vi "GOOP_LVClass_Item_OnCommand.vi"(10 "Command Tag":string, 11 "Object":u64) -> ()   [LabVIEW 2020]
uses:
  <resource>/Framework/Providers/Open_GDS/SubVIs/GOOP_ClassProviderClassType.ctl
  <resource>/Framework/Providers/Open_GDS/ClassProviders/Provider_BaseClassInterface/ClassWriter_class/ClassWriter.lvclass
  <resource>/Framework/Providers/Open_GDS/ClassProviders/Common/ScriptingFunctions/Scripting_ConnectorPanePatternType.ctl
  <resource>/Framework/Providers/Open_GDS/SubVIs/GOOP_UMLEditor_CallMainAction.ctl
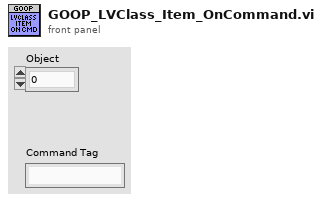
[diagram p1: front panel]
types:
  T1 = typedef "GOOP_ClassProviderClassType.ctl" = enum16{"ClassWriter", "ClassReader"}
  T2 = typedef "GOOP_UMLEditor_CallMainAction.ctl" = enum16{"OpenUmlEditor", "ReverseEngineering:WholeProject", "ReverseEngineering:OneClass", "ReverseEngineering:OneVI", "ShowInStateDiagram:OneVI", "OpenUMLFile"}
  T3 = enum8{"No dynamic dispatch VIs", "Include nearest implementation", "Include all overrides"}
  T4 = typedef "Scripting_ConnectorPanePatternType.ctl" = u16
  T5 = typedef "GDSLvCLass_ClassSettingsType.ctl" = cluster{"ClassProviderName":string, "ClassTemplateUsed":string, "ClassTemplateVersion":string, "ClassDescription":string, "PlugIns":T6[], "ConnectorPanePattern":string}
  T6 = typedef "GDSLvClass_PlugIn.ctl" = cluster{"Type":T7, "ID":string, "Version":string, "Path":path, "Name":string, "Data":variant}
  T7 = typedef "GDSLvClass_PlugInTypes.ctl" = enum16{"DesignPattern", "MethodTypes"}
  T8 = typedef "AddDesignPatternData.ctl" = cluster{"Type":string, "ID":string, "Version":string, "VIPath":path, "Name":string, "Data":variant}
  T9 = typedef "ClassWriter.lvclass/CreateMethodData.ctl" = cluster{"MethodName":string, "RelativeMethodPath":path, "MethodDescription":string, "Scope/Visibility":T10, "MethodTemplateName":string, "IconOut":u8[][], "RelativeProjectClassPath":string, "OpenViAfterCreation":bool, "DynamicDispatchVi":bool, "ExtraCreateParameters":variant, "MustOverride":bool, "MustCallParent":bool, "IconDetails":T11, "AF-Option":variant, "TemplatePath":path}
  T10 = typedef "GOOP300_MethodScopeType.ctl" = enum16{"Use Parent Folder Scope", "Public", "Protected", "Private", "Community"}
  T11 = typedef "ClassWriterNative.lvclass/IconDetails.ctl" = cluster{"IconSize":T12, "ImageRows(32)":i32, "ConnectorPaneHeight":i32[]}
  T12 = typedef "ClassWriterNative.lvclass/IconSize.ctl" = enum16{"Full", "1 c-term high", "2 c-term high", "3 c-term high"}
  T13 = typedef "ClassWriter.lvclass/CreateClassData.ctl" = cluster{"ClassName":string, "ClassFolder":path, "ClassDescription":string, "ClassTemplateOptions":string, "BaseClass(ProjectStringPath or LvClassFilePath)":variant, "ExtraCreateParameters":variant, "FolderSuffix":string, "ParentInterfaces":path[]}
  T14 = typedef "ItemRef.ctl" = u64
  T15 = typedef "ClassWriter.lvclass/HandleInterfacesData.ctl" = cluster{"InterfaceToAdd(Path)":path[], "InterfaceToRemove(Path)":path[], "MethodsToAddPerInterface(Empty=>All)":cluster{"InterfacePath":path, "Methods":string[]}[], "MethodsToRemovePerInterface(Empty=>All)":cluster{"InterfacePath":path, "Methods":string[]}[]}
  T16 = enum32{"invalid scope", "public", "private", "protected", "community"}
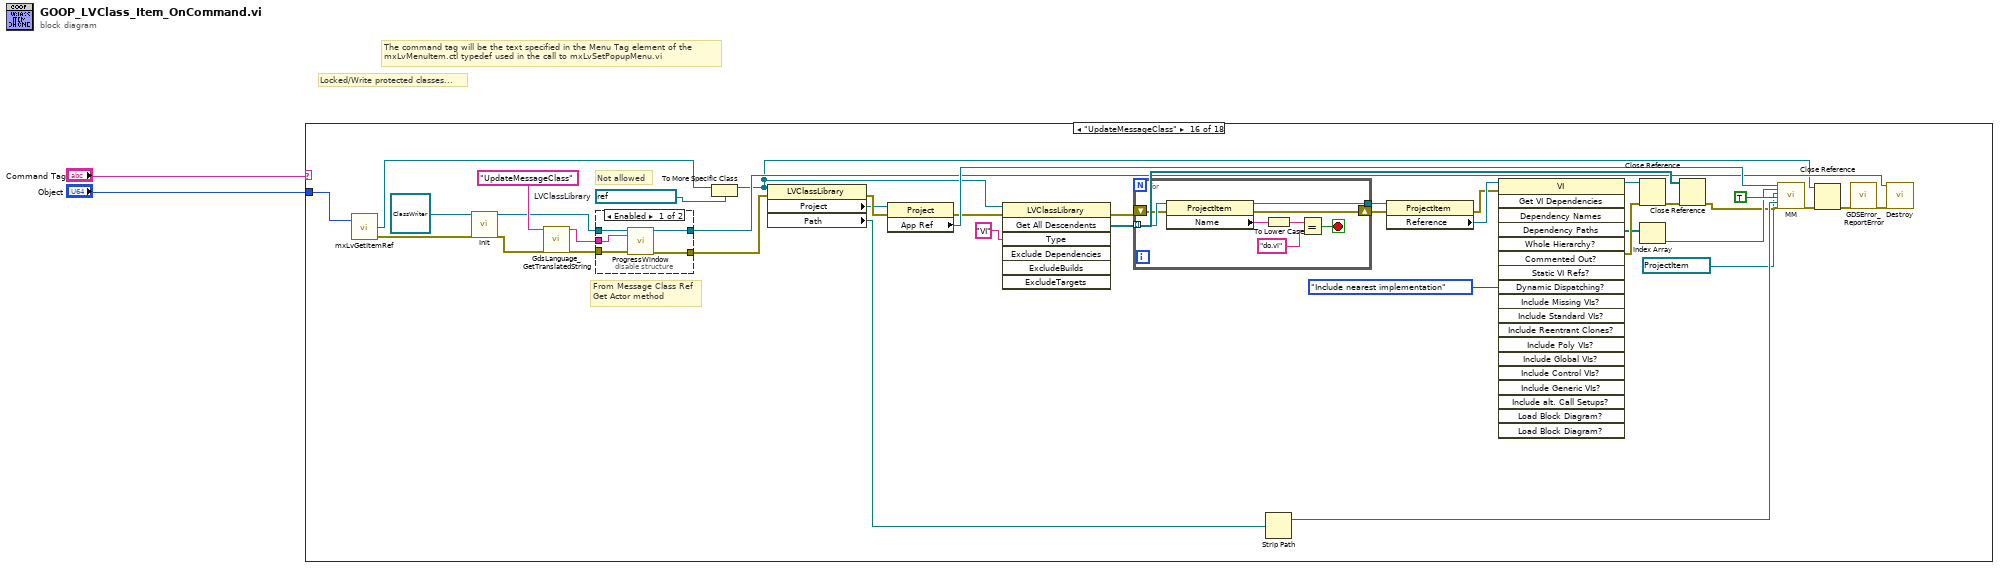
[diagram p0: block diagram]
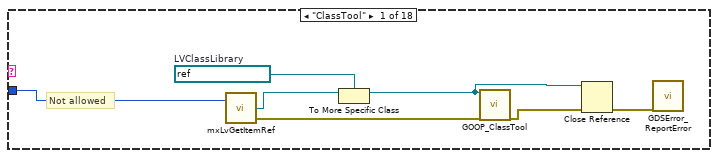
[diagram p2: hidden frame]
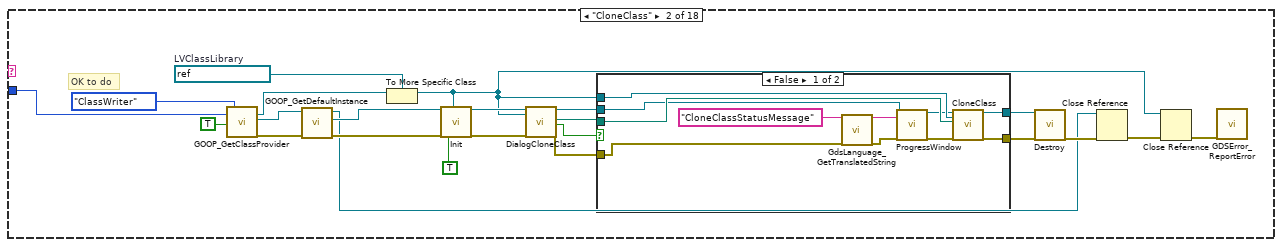
[diagram p3: hidden frame]
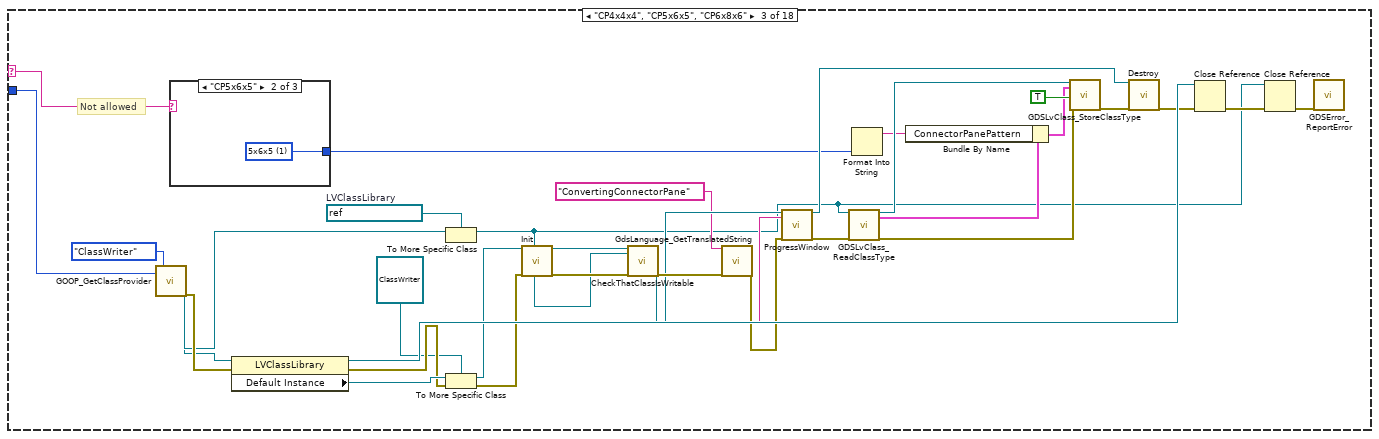
[diagram p5: hidden frame]
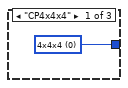
[diagram p6: hidden frame]
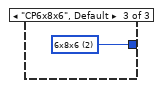
[diagram p7: hidden frame]
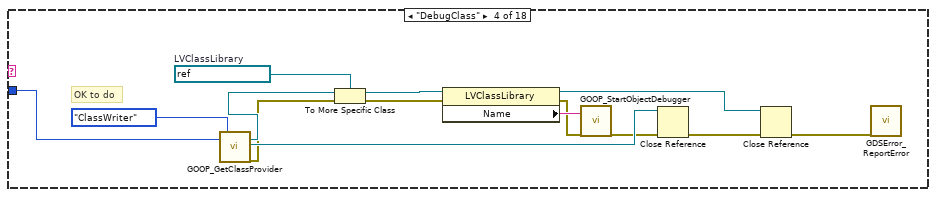
[diagram p8: hidden frame]
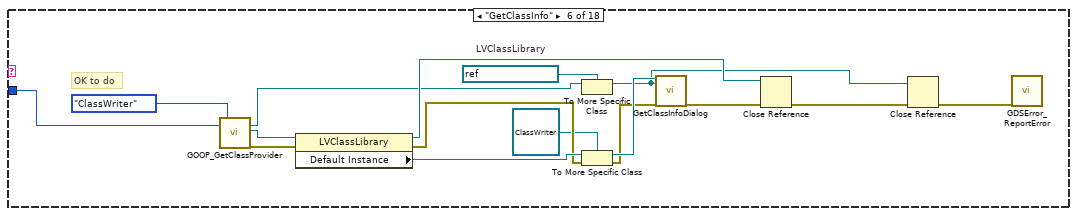
[diagram p10: hidden frame]
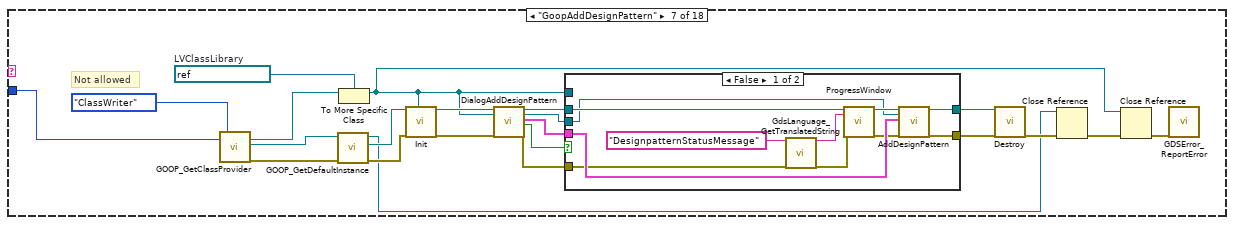
[diagram p11: hidden frame]
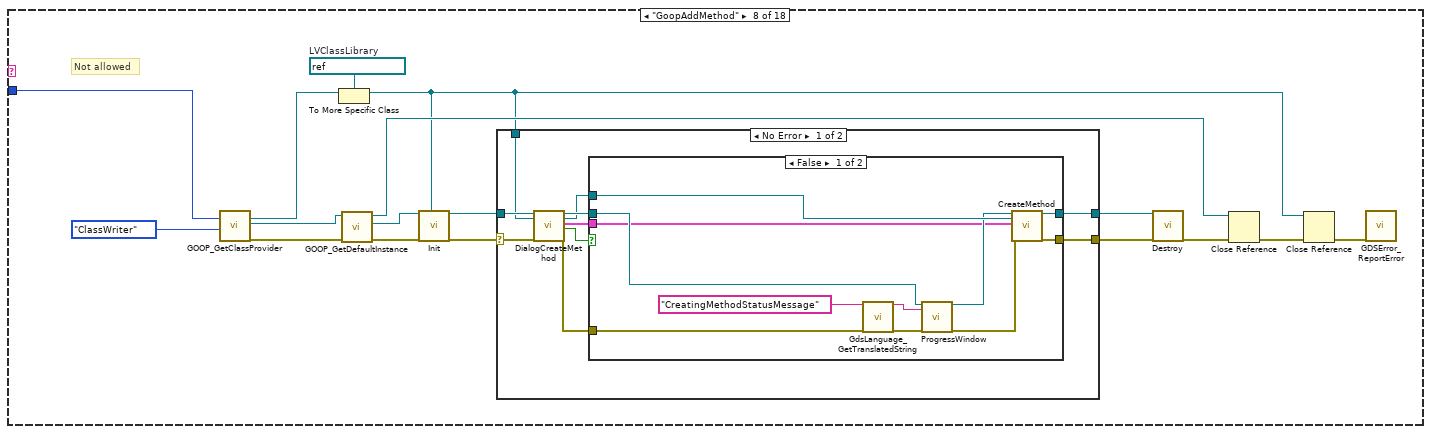
[diagram p13: hidden frame]
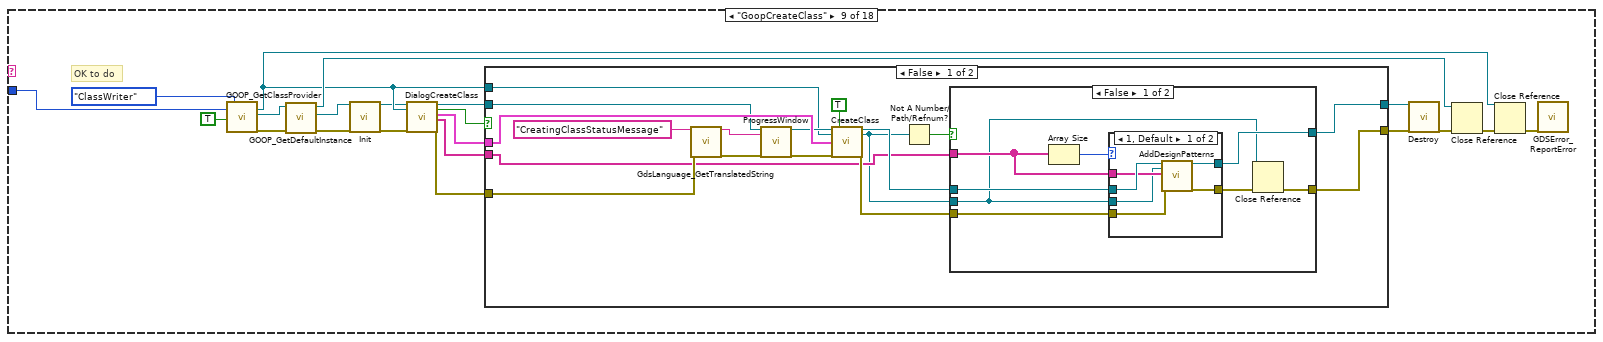
[diagram p16: hidden frame]
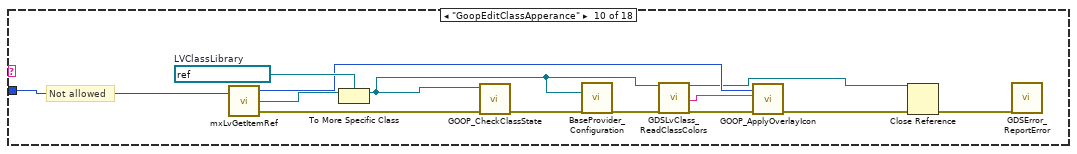
[diagram p20: hidden frame]
diagram:
  # "Locked/Write protected classes..."
  # "The command tag will be the text specified in the Menu Tag element of the \nmxLvMenuItem.ctl typedef used in the call to mxLvSetPopupMenu.vi"
  n1 = case shown="\"UpdateMessageClass\"" "Command Tag" {
    selector: "Command Tag" -> [_ _ w46 _ _ _ _ _ _ _ _ _ _ _ _ _ _ w522]
    tunnel: "Object" -> [w8 w19 w66 w83 _ w112 w134 w164 w210 w258 w268 w285 w323 w347 w373 w451 w470 w523]
    frame "ClassTool" {
      w9 = refnum<vi> refnum  # LVClassLibrary
      # "Not allowed"
      n2 = call <resource>:"mxLvGetItemRef.vi"("Item"=w8) -> ("Item Refnum"=w7:refnum<vi>, "error out"=w5:errorcluster)  [unwired: 1 in, 1 out]
      n3 = To More Specific Class(target class=w9, reference=w7) -> (specific class reference=w4:refnum<vi>)  [unwired: 1 in, 1 out]
      n4 = call <resource>:"GOOP_ClassTool.vi"("ClassRef"=w4, "Error In"=w5) -> ("Error Out"=w3:errorcluster)  [unwired: 17 in]
      n5 = Close Reference(reference=w4, error in (no error)=w3) -> (error out=w6:errorcluster)
      n6 = call <resource>:"GDSError_ReportError.vi"("error in (no error)"=w6) -> ()  [unwired: 18 in, 1 out]
    }
    frame "CloneClass" {
      w29 = refnum<vi> refnum  # LVClassLibrary
      # "OK to do"
      n7 = call <resource>:"GOOP_GetClassProvider.vi"("New Item Parent/Object"=w19, "CreateClass"=TRUE, "ProviderClassType"=GOOP_ClassProviderClassType."ClassWriter") -> ("ProjectItem"=w30:refnum<vi>, "LVClass.Open"=w16:refnum<vi>, "error out"=w17:errorcluster)  [unwired: 14 in]
      n8 = call <resource>:"GOOP_GetDefaultInstance.vi"("error in"=w17, "LVClassIn"=w16) -> ("error out"=w14:errorcluster, "ClassWriter.lvclass"=w15:refnum<class "ClassWriter.lvclass">, "LVClassOut"=w13:refnum<vi>)  [unwired: 7 in]
      n9 = To More Specific Class(target class=w29, reference=w30) -> (specific class reference=w10:refnum<vi>)  [unwired: 1 in, 1 out]
      n10 = call-dynamic "Init.vi"("ClassWriter in"=w15, "error in (no error)"=w14, "ClassFileMayBeReadOnly(False)"=TRUE, "LVClassLibrary Refnum"=w10) -> ("ClassWriter out"=w22:refnum<class "ClassWriter.lvclass">, "error out"=w21:errorcluster)  [unwired: 14 in]
      n11 = call-dynamic "DialogCloneClass.vi"("ClassWriter.lvclass"=w22, "ClassItemRefIn"=w10, "error in (no error)"=w21) -> ("ClassWriter.lvclassOut"=w27:refnum<class "ClassWriter.lvclass">, "NewClassPath"=w23:path, "Cancelled"=w24:bool, "error out"=w26:errorcluster)  [unwired: 12 in, 1 out]
      n12 = case shown="False" w24 {
        tunnel: w27 -> [w35 w44]
        tunnel: w26 -> [w36 w45]
        tunnel: [w40 w45] -> w25
        tunnel: w10 -> [w43 _]
        tunnel: w23 -> [w42 _]
        tunnel: [w41 w44] -> w20
        frame False {
          n13 = call <resource>:"GdsLanguage_GetTranslatedString.vi"("StringID(s)"="CloneClassStatusMessage" ("Message(Exit)"), "error in (no error)"=w36) -> ("FirstStringOut"=w37:string, "error out"=w38:errorcluster)  [unwired: 14 in, 2 out]
          n14 = call-dynamic "ProgressWindow.vi"("ClassWriter in"=w35, "Message(Exit)"=w37, "error in (no error)"=w38) -> ("ClassWriter out"=w34:refnum<class "ClassWriter.lvclass">, "error out"=w33:errorcluster)  [unwired: 15 in]
          n15 = call-dynamic "CloneClass.vi"("ClassWriter.lvclass"=w34, "ClassRef"=w43, "NewClassPath"=w42, "error in (no error)"=w33) -> ("ClassWriter.lvclass"=w41:refnum<class "ClassWriter.lvclass">, "error out"=w40:errorcluster)  [unwired: 13 in, 1 out]
        }
        frame True {
        }
      }
      n16 = call-dynamic "Destroy.vi"("ClassWriter.lvclass"=w20, "error in (no error)"=w25) -> ("error out"=w28:errorcluster)  [unwired: 17 in]
      n17 = Close Reference(reference=w13, error in (no error)=w28) -> (error out=w32:errorcluster)
      n18 = Close Reference(reference=w10, error in (no error)=w32) -> (error out=w18:errorcluster)
      n19 = call <resource>:"GDSError_ReportError.vi"("error in (no error)"=w18) -> ()  [unwired: 18 in, 1 out]
    }
    frame "CP4x4x4", "CP5x6x5", "CP6x8x6" {
      w72 = refnum<vi> refnum  # LVClassLibrary
      # "Not allowed"
      n20 = call <resource>:"GOOP_GetClassProvider.vi"("New Item Parent/Object"=w66, "ProviderClassType"=GOOP_ClassProviderClassType."ClassWriter") -> ("ProjectItem"=w73:refnum<vi>, "LVClass.Open"=w71:refnum<vi>, "error out"=w76:errorcluster)  [unwired: 15 in]
      n21 = case shown="\"CP5x6x5\"" w46 {
        tunnel: [w80 w81 w82] -> w48
        frame "CP4x4x4" {
          w80 = T4 0 items=["4x4x4", "5x6x5", "6x8x6"] ("Pattern")
        }
        frame "CP5x6x5" {
          w81 = T4 1 items=["4x4x4", "5x6x5", "6x8x6"] ("Pattern")
        }
        frame "CP6x8x6", Default {
          w82 = T4 2 items=["4x4x4", "5x6x5", "6x8x6"] ("Pattern")
        }
      }
      n22 = property class="LVClassLibrary"(reference=w71, error in=w76) -> (reference out=w74:refnum<vi>, error out=w78:errorcluster, "Default Instance"=w79:refnum<class>)
      n23 = To More Specific Class(target class=w72, reference=w73) -> (specific class reference=w52:refnum<vi>)  [unwired: 1 in, 1 out]
      n24 = To More Specific Class(target class=refnum<class "ClassWriter.lvclass"> refnum ("ClassWriter.lvclass"), reference=w79, error in=w78) -> (specific class reference=w67:refnum<class "ClassWriter.lvclass">, error out=w68:errorcluster)
      n25 = call-dynamic "Init.vi"("ClassWriter in"=w67, "error in (no error)"=w68, "LVClassLibrary Refnum"=w52) -> ("ClassWriter out"=w64:refnum<class "ClassWriter.lvclass">, "error out"=w63:errorcluster)  [unwired: 15 in]
      n26 = call <resource>:"CheckThatClassIsWritable.vi"("ClassWriter in"=w64, "Library Refnum"=w52, "error in (no error)"=w63) -> ("ClassWriter out"=w61:refnum<class "ClassWriter.lvclass">, "error out"=w62:errorcluster)  [unwired: 15 in]
      n27 = call <resource>:"GdsLanguage_GetTranslatedString.vi"("StringID(s)"="ConvertingConnectorPane" ("Message(Exit)"), "error in (no error)"=w62) -> ("FirstStringOut"=w58:string, "error out"=w60:errorcluster)  [unwired: 14 in, 2 out]
      n28 = call-dynamic "ProgressWindow.vi"("ClassWriter in"=w61, "Message(Exit)"=w58, "error in (no error)"=w60) -> ("ClassWriter out"=w57:refnum<class "ClassWriter.lvclass">, "error out"=w56:errorcluster)  [unwired: 15 in]
      n29 = call <resource>:"GDSLvClass_ReadClassType.vi"("Class Refnum In"=w52, "error in (no error)"=w56) -> ("Class Refnum Out"=w55:refnum<vi>, "ClassSettings"=w54:T5, "error out"=w53:errorcluster)  [unwired: 15 in]
      n30 = Format Into String(w48) -> (resulting string=w47:string)  [unwired: 3 in, 1 out]
      n31 = Bundle By Name(cluster=w54, "ConnectorPanePattern"=w47) -> (w49:T5)
      n32 = call <resource>:"GDSLvClass_StoreClassType.vi"("Class Refnum In"=w55, "ClassSettings"=w49, "CheckAndFixConnectorPaneType(False)"=TRUE, "error in (no error)"=w53) -> ("error out"=w51:errorcluster)  [unwired: 14 in, 1 out]
      n33 = call-dynamic "Destroy.vi"("ClassWriter.lvclass"=w57, "error in (no error)"=w51) -> ("error out"=w70:errorcluster)  [unwired: 17 in]
      n34 = Close Reference(reference=w74, error in (no error)=w70) -> (error out=w77:errorcluster)
      n35 = Close Reference(reference=w52, error in (no error)=w77) -> (error out=w65:errorcluster)
      n36 = call <resource>:"GDSError_ReportError.vi"("error in (no error)"=w65) -> ()  [unwired: 18 in, 1 out]
    }
    frame "DebugClass" {
      w92 = refnum<vi> refnum  # LVClassLibrary
      # "OK to do"
      n37 = call <resource>:"GOOP_GetClassProvider.vi"("New Item Parent/Object"=w83, "ProviderClassType"=GOOP_ClassProviderClassType."ClassWriter") -> ("ProjectItem"=w93:refnum<vi>, "LVClass.Open"=w91:refnum<vi>, "error out"=w84:errorcluster)  [unwired: 15 in]
      n38 = To More Specific Class(target class=w92, reference=w93, error in=w84) -> (specific class reference=w90:refnum<vi>, error out=w85:errorcluster)
      n39 = property class="LVClassLibrary"(reference=w90, error in=w85) -> (reference out=w89:refnum<vi>, error out=w86:errorcluster, "Name"=w88:string)
      n40 = call <resource>:"GOOP_StartObjectDebugger.vi"("ClassToOpen"=w88, "error in (no error)"=w86) -> ("error out"=w87:errorcluster)  [unwired: 17 in]
      n41 = Close Reference(reference=w91, error in (no error)=w87) -> (error out=w96:errorcluster)
      n42 = Close Reference(reference=w89, error in (no error)=w96) -> (error out=w95:errorcluster)
      n43 = call <resource>:"GDSError_ReportError.vi"("error in (no error)"=w95) -> ()  [unwired: 18 in, 1 out]
    }
    frame "False" {
    }
    frame "GetClassInfo" {
      w101 = refnum<vi> refnum  # LVClassLibrary
      # "OK to do"
      n44 = call <resource>:"GOOP_GetClassProvider.vi"("New Item Parent/Object"=w112, "ProviderClassType"=GOOP_ClassProviderClassType."ClassWriter") -> ("ProjectItem"=w102:refnum<vi>, "LVClass.Open"=w107:refnum<vi>, "error out"=w106:errorcluster)  [unwired: 15 in]
      n45 = property class="LVClassLibrary"(reference=w107, error in=w106) -> (reference out=w104:refnum<vi>, error out=w110:errorcluster, "Default Instance"=w111:refnum<class>)
      n46 = To More Specific Class(target class=w101, reference=w102) -> (specific class reference=w97:refnum<vi>)  [unwired: 1 in, 1 out]
      n47 = To More Specific Class(target class=refnum<class "ClassWriter.lvclass"> refnum ("ClassWriter.lvclass"), reference=w111, error in=w110) -> (specific class reference=w100:refnum<class "ClassWriter.lvclass">, error out=w99:errorcluster)
      n48 = call-dynamic "GetClassInfoDialog.vi"("ClassWriter in"=w100, "ClassItemRefIn"=w97, "error in (no error)"=w99) -> ("error out"=w98:errorcluster)  [unwired: 15 in, 1 out]
      n49 = Close Reference(reference=w104, error in (no error)=w98) -> (error out=w109:errorcluster)
      n50 = Close Reference(reference=w97, error in (no error)=w109) -> (error out=w108:errorcluster)
      n51 = call <resource>:"GDSError_ReportError.vi"("error in (no error)"=w108) -> ()  [unwired: 18 in, 1 out]
    }
    frame "GoopAddDesignPattern" {
      w126 = refnum<vi> refnum  # LVClassLibrary
      # "Not allowed"
      n52 = call <resource>:"GOOP_GetClassProvider.vi"("New Item Parent/Object"=w134, "ProviderClassType"=GOOP_ClassProviderClassType."ClassWriter") -> ("ProjectItem"=w127:refnum<vi>, "LVClass.Open"=w115:refnum<vi>, "error out"=w114:errorcluster)  [unwired: 15 in]
      n53 = call <resource>:"GOOP_GetDefaultInstance.vi"("error in"=w114, "LVClassIn"=w115) -> ("error out"=w118:errorcluster, "ClassWriter.lvclass"=w117:refnum<class "ClassWriter.lvclass">, "LVClassOut"=w116:refnum<vi>)  [unwired: 7 in]
      n54 = To More Specific Class(target class=w126, reference=w127) -> (specific class reference=w113:refnum<vi>)  [unwired: 1 in, 1 out]
      n55 = call-dynamic "Init.vi"("ClassWriter in"=w117, "error in (no error)"=w118, "LVClassLibrary Refnum"=w113) -> ("ClassWriter out"=w119:refnum<class "ClassWriter.lvclass">, "error out"=w120:errorcluster)  [unwired: 15 in]
      n56 = call-dynamic "DialogAddDesignPattern.vi"("ClassWriter in"=w119, "ClassItemRefIn"=w113, "error in (no error)"=w120) -> ("ClassWriter out"=w130:refnum<class "ClassWriter.lvclass">, "ClassItemRefOut"=w129:refnum<vi>, "CreateMethodData"=w125:T8, "Cancelled"=w124:bool, "error out"=w128:errorcluster)  [unwired: 12 in]
      n57 = case shown="False" w124 {
        tunnel: w130 -> [w138 w146]
        tunnel: w129 -> [w135 _]
        tunnel: w128 -> [w140 w147]
        tunnel: w113 -> [_ _]
        tunnel: [w144 w147] -> w123
        tunnel: w125 -> [w145 _]
        tunnel: [w136 w146] -> w122
        frame False {
          n58 = call <resource>:"GdsLanguage_GetTranslatedString.vi"("StringID(s)"="DesignpatternStatusMessage" ("Message(Exit)"), "error in (no error)"=w140) -> ("FirstStringOut"=w143:string, "error out"=w142:errorcluster)  [unwired: 14 in, 2 out]
          n59 = call-dynamic "ProgressWindow.vi"("ClassWriter in"=w138, "Message(Exit)"=w143, "error in (no error)"=w142) -> ("ClassWriter out"=w137:refnum<class "ClassWriter.lvclass">, "error out"=w139:errorcluster)  [unwired: 15 in]
          n60 = call-dynamic "AddDesignPattern.vi"("ClassWriter.lvclass"=w137, "ClassItemRefIn"=w135, "AddDesignPatternData"=w145, "error in (no error)"=w139) -> ("ClassWriter.lvclass"=w136:refnum<class "ClassWriter.lvclass">, "error out"=w144:errorcluster)  [unwired: 13 in, 1 out]
        }
        frame True {
        }
      }
      n61 = call-dynamic "Destroy.vi"("ClassWriter.lvclass"=w122, "error in (no error)"=w123) -> ("error out"=w121:errorcluster)  [unwired: 17 in]
      n62 = Close Reference(reference=w116, error in (no error)=w121) -> (error out=w133:errorcluster)
      n63 = Close Reference(reference=w113, error in (no error)=w133) -> (error out=w132:errorcluster)
      n64 = call <resource>:"GDSError_ReportError.vi"("error in (no error)"=w132) -> ()  [unwired: 18 in, 1 out]
    }
    frame "GoopAddMethod" {
      w159 = refnum<vi> refnum  # LVClassLibrary
      # "Not allowed"
      n65 = call <resource>:"GOOP_GetClassProvider.vi"("New Item Parent/Object"=w164, "ProviderClassType"=GOOP_ClassProviderClassType."ClassWriter") -> ("ProjectItem"=w160:refnum<vi>, "LVClass.Open"=w150:refnum<vi>, "error out"=w149:errorcluster)  [unwired: 15 in]
      n66 = To More Specific Class(target class=w159, reference=w160) -> (specific class reference=w148:refnum<vi>)  [unwired: 1 in, 1 out]
      n67 = call <resource>:"GOOP_GetDefaultInstance.vi"("error in"=w149, "LVClassIn"=w150) -> ("error out"=w153:errorcluster, "ClassWriter.lvclass"=w152:refnum<class "ClassWriter.lvclass">, "LVClassOut"=w151:refnum<vi>)  [unwired: 7 in]
      n68 = call-dynamic "Init.vi"("ClassWriter in"=w152, "error in (no error)"=w153, "LVClassLibrary Refnum"=w148) -> ("ClassWriter out"=w154:refnum<class "ClassWriter.lvclass">, "error out"=w155:errorcluster)  [unwired: 15 in]
      n69 = case shown="No Error" w155 {
        selector: w155 -> [w167 w189]
        tunnel: [w169 w189] -> w158
        tunnel: [w168 w188] -> w157
        tunnel: w154 -> [w166 w188]
        tunnel: w148 -> [w165 _]
        frame No Error {
          n70 = call-dynamic "DialogCreateMethod.vi"("ClassWriter in"=w166, "ClassItemRefIn"=w165, "error in (no error)"=w167) -> ("ClassWriter out"=w174:refnum<class "ClassWriter.lvclass">, "ClassItemRefOut"=w173:refnum<vi>, "CreateMethodData"=w171:T9, "Cancelled"=w170:bool, "error out"=w172:errorcluster)  [unwired: 12 in]
          n71 = case shown="False" w170 {
            tunnel: w174 -> [w178 w186]
            tunnel: w173 -> [w185 _]
            tunnel: w172 -> [w180 w187]
            tunnel: [w184 w187] -> w169
            tunnel: w171 -> [w175 _]
            tunnel: [w176 w186] -> w168
            frame False {
              n72 = call <resource>:"GdsLanguage_GetTranslatedString.vi"("StringID(s)"="CreatingMethodStatusMessage" ("Message(Exit)"), "error in (no error)"=w180) -> ("FirstStringOut"=w183:string, "error out"=w182:errorcluster)  [unwired: 14 in, 2 out]
              n73 = call-dynamic "ProgressWindow.vi"("ClassWriter in"=w178, "Message(Exit)"=w183, "error in (no error)"=w182) -> ("ClassWriter out"=w177:refnum<class "ClassWriter.lvclass">, "error out"=w179:errorcluster)  [unwired: 15 in]
              n74 = call-dynamic "CreateMethod.vi"("ClassWriter.lvclass"=w177, "ClassItemRefIn"=w185, "CreateMethodData"=w175, "error in (no error)"=w179) -> ("ClassWriter.lvclass"=w176:refnum<class "ClassWriter.lvclass">, "error out"=w184:errorcluster)  [unwired: 12 in, 2 out]
            }
            frame True {
            }
          }
        }
        frame Error {
        }
      }
      n75 = call-dynamic "Destroy.vi"("ClassWriter.lvclass"=w157, "error in (no error)"=w158) -> ("error out"=w156:errorcluster)  [unwired: 17 in]
      n76 = Close Reference(reference=w151, error in (no error)=w156) -> (error out=w163:errorcluster)
      n77 = Close Reference(reference=w148, error in (no error)=w163) -> (error out=w162:errorcluster)
      n78 = call <resource>:"GDSError_ReportError.vi"("error in (no error)"=w162) -> ()  [unwired: 18 in, 1 out]
    }
    frame "GoopCreateClass" {
      # "OK to do"
      n79 = call <resource>:"GOOP_GetClassProvider.vi"("New Item Parent/Object"=w210, "CreateClass"=TRUE, "ProviderClassType"=GOOP_ClassProviderClassType."ClassWriter") -> ("ProjectItem"=w199:refnum<vi>, "LVClass.Open"=w207:refnum<vi>, "error out"=w206:errorcluster)  [unwired: 14 in]
      n80 = call <resource>:"GOOP_GetDefaultInstance.vi"("error in"=w206, "LVClassIn"=w207) -> ("error out"=w191:errorcluster, "ClassWriter.lvclass"=w192:refnum<class "ClassWriter.lvclass">, "LVClassOut"=w202:refnum<vi>)  [unwired: 7 in]
      n81 = call-dynamic "Init.vi"("ClassWriter in"=w192, "error in (no error)"=w191) -> ("ClassWriter out"=w194:refnum<class "ClassWriter.lvclass">, "error out"=w193:errorcluster)  [unwired: 16 in]
      n82 = call-dynamic "DialogCreateClass.vi"("ClassWriter in"=w194, "ProjectItem Refnum"=w199, "error in (no error)"=w193) -> ("ClassWriter out"=w204:refnum<class "ClassWriter.lvclass">, "Cancelled"=w200:bool, "CreateClassData"=w201:T13, "DesignPatternsToAddAfterCreation"=w190:string[], "error out"=w203:errorcluster)  [unwired: 10 in, 2 out]
      n83 = case shown="False" w200 {
        tunnel: w204 -> [w222 w246]
        tunnel: w203 -> [w223 w247]
        tunnel: w199 -> [w215 _]
        tunnel: [w213 w247] -> w198
        tunnel: w201 -> [w227 _]
        tunnel: [w217 w246] -> w196
        tunnel: w190 -> [w216 _]
        frame False {
          n84 = call <resource>:"GdsLanguage_GetTranslatedString.vi"("StringID(s)"="CreatingClassStatusMessage" ("Message(Exit)"), "error in (no error)"=w223) -> ("FirstStringOut"=w224:string, "error out"=w225:errorcluster)  [unwired: 14 in, 2 out]
          n85 = call-dynamic "ProgressWindow.vi"("ClassWriter in"=w222, "Message(Exit)"=w224, "error in (no error)"=w225) -> ("ClassWriter out"=w221:refnum<class "ClassWriter.lvclass">, "error out"=w220:errorcluster)  [unwired: 15 in]
          n86 = call-dynamic "CreateClass.vi"("ClassWriter.lvclass"=w221, "ProjectTreePosition(String or Project Item Ref)"=w215, "CreateClassData"=w227, "error in (no error)"=w220, "KeepLvClassRefOpen(False)"=TRUE) -> ("ClassWriter.lvclass"=w219:refnum<class "ClassWriter.lvclass">, "LVClassLibraryRefnum"=w212:refnum<vi>, "error out"=w218:errorcluster)  [unwired: 11 in, 1 out]
          n87 = Not A Number/Path/Refnum?(number/path/refnum=w212) -> (NaN/Path/Refnum?=w211:bool)
          n88 = case shown="False" w211 {
            tunnel: w219 -> [w234 w245]
            tunnel: w218 -> [w233 w244]
            tunnel: [w232 w245] -> w217
            tunnel: w216 -> [w231 _]
            tunnel: [w229 w244] -> w213
            tunnel: w212 -> [w228 _]
            frame False {
              n89 = Array Size(array=w231) -> (size(s)=w235:i32)
              n90 = case shown="1, Default" w235 {
                tunnel: w234 -> [w241 w243]
                tunnel: w233 -> [w240 w242]
                tunnel: [w239 w242] -> w230
                tunnel: [w238 w243] -> w232
                tunnel: w231 -> [w237 _]
                tunnel: w228 -> [w236 _]
                frame 1, Default {
                  n91 = call-dynamic "AddDesignPatterns.vi"("ClassWriterNative"=w241, "ClassItemRefIn"=w236, "DesignPatterns"=w237, "error in (no error)"=w240) -> ("ClassWriterNative"=w238:refnum<class "ClassWriter.lvclass">, "error out"=w239:errorcluster)  [unwired: 12 in, 2 out]
                }
                frame 0 {
                }
              }
              n92 = Close Reference(reference=w228, error in (no error)=w230) -> (error out=w229:errorcluster)
            }
            frame True {
            }
          }
        }
        frame True {
        }
      }
      n93 = call-dynamic "Destroy.vi"("ClassWriter.lvclass"=w196, "error in (no error)"=w198) -> ("error out"=w197:errorcluster)  [unwired: 17 in]
      n94 = Close Reference(reference=w202, error in (no error)=w197) -> (error out=w209:errorcluster)
      n95 = Close Reference(reference=w199, error in (no error)=w209) -> (error out=w208:errorcluster)
      n96 = call <resource>:"GDSError_ReportError.vi"("error in (no error)"=w208) -> ()  [unwired: 18 in, 1 out]
    }
    frame "GoopEditClassApperance" {
      w260 = refnum<vi> refnum  # LVClassLibrary
      # "Not allowed"
      n97 = call <resource>:"mxLvGetItemRef.vi"("Item"=w258) -> ("Item"=w256:T14, "Item Refnum"=w259:refnum<vi>, "error out"=w250:errorcluster)  [unwired: 1 in]
      n98 = To More Specific Class(target class=w260, reference=w259) -> (specific class reference=w248:refnum<vi>)  [unwired: 1 in, 1 out]
      n99 = call <resource>:"GOOP_CheckClassState.vi"("error in"=w250, "Library Refnum"=w248) -> ("error out"=w249:errorcluster)  [unwired: 9 in]
      n100 = call <resource>:"BaseProvider_Configuration.vi"("ClassRef/ClassPath(If empty Configuration default will be modified)"=w248, "Error In"=w249) -> ("Error Out"=w255:errorcluster)  [unwired: 16 in, 1 out]
      n101 = call <resource>:"GDSLvClass_ReadClassColors.vi"("Library Refnum"=w248, "error in (no error)"=w255) -> ("Library Refnum"=w252:refnum<vi>, "ClassItemIconName(NoExtension)"=w257:string, "error out"=w254:errorcluster)  [unwired: 12 in, 3 out]
      n102 = call <resource>:"GOOP_ApplyOverlayIcon.vi"("error in (no error)"=w254, "IconName(NoPngExtension)"=w257, "Object"=w256) -> ("error out"=w253:errorcluster)  [unwired: 8 in]
      n103 = Close Reference(reference=w252, error in (no error)=w253) -> (error out=w251:errorcluster)
      n104 = call <resource>:"GDSError_ReportError.vi"("error in (no error)"=w251) -> ()  [unwired: 18 in, 1 out]
    }
    frame "GoopEditClassIcon" {
      w269 = refnum<vi> refnum  # LVClassLibrary
      # "Not allowed"
      n105 = call <resource>:"mxLvGetItemRef.vi"("Item"=w268) -> ("Item Refnum"=w267:refnum<vi>, "error out"=w262:errorcluster)  [unwired: 1 in, 1 out]
      n106 = To More Specific Class(target class=w269, reference=w267) -> (specific class reference=w261:refnum<vi>)  [unwired: 1 in, 1 out]
      n107 = call <resource>:"GOOP_CheckClassState.vi"("error in"=w262, "Library Refnum"=w261) -> ("error out"=w263:errorcluster)  [unwired: 9 in]
      n108 = call <resource>:"CheckThatClassIsWritable.vi"("Library Refnum"=w261, "error in (no error)"=w263) -> ("error out"=w264:errorcluster)  [unwired: 16 in, 1 out]
      n109 = call <resource>:"GDSLvIcon_DialogUpdateClass.vi"("ClassPath(FilePath/ProjectTreePath/LvCLassRef)"=w261, "error in (no error)"=w264) -> ("error out"=w266:errorcluster)  [unwired: 13 in, 4 out]
      n110 = Close Reference(reference=w261, error in (no error)=w266) -> (error out=w265:errorcluster)
      n111 = call <resource>:"GDSError_ReportError.vi"("error in (no error)"=w265) -> ()  [unwired: 18 in, 1 out]
    }
    frame "ManageInterfaces" {
      w289 = refnum<vi> refnum  # LVClassLibrary
      # "OK to do"
      n112 = call <resource>:"GOOP_GetClassProvider.vi"("New Item Parent/Object"=w285, "CreateClass"=TRUE, "ProviderClassType"=GOOP_ClassProviderClassType."ClassWriter") -> ("ProjectItem"=w290:refnum<vi>, "LVClass.Open"=w282:refnum<vi>, "error out"=w283:errorcluster)  [unwired: 14 in]
      n113 = To More Specific Class(target class=w289, reference=w290) -> (specific class reference=w271:refnum<vi>)  [unwired: 1 in, 1 out]
      n114 = call <resource>:"GOOP_GetDefaultInstance.vi"("error in"=w283, "LVClassIn"=w282) -> ("error out"=w280:errorcluster, "ClassWriter.lvclass"=w281:refnum<class "ClassWriter.lvclass">, "LVClassOut"=w279:refnum<vi>)  [unwired: 7 in]
      n115 = call-dynamic "Init.vi"("ClassWriter in"=w281, "error in (no error)"=w280, "ClassFileMayBeReadOnly(False)"=TRUE, "LVClassLibrary Refnum"=w271) -> ("ClassWriter out"=w276:refnum<class "ClassWriter.lvclass">, "error out"=w275:errorcluster)  [unwired: 14 in]
      n116 = call-dynamic "DialogManageInterfaces.vi"("error in (no error)"=w275, "ClassItemRefIn"=w271, "ClassWriterIn"=w276) -> ("error out"=w273:errorcluster, "HandleInterfacesData"=w270:T15, "Cancelled"=w274:bool, "ClassWriterOut"=w272:refnum<class "ClassWriter.lvclass">)  [unwired: 5 in]
      n117 = case shown="False" w274 {
        tunnel: w272 -> [w301 w302]
        tunnel: w273 -> [w299 w303]
        tunnel: [w296 w303] -> w287
        tunnel: w271 -> [w294 _]
        tunnel: [w295 w302] -> w286
        tunnel: w270 -> [w293 _]
        frame False {
          n118 = call-dynamic "ProgressWindow.vi"("ClassWriter in"=w301, "Message(Exit)"="Updating", "error in (no error)"=w299) -> ("ClassWriter out"=w298:refnum<class "ClassWriter.lvclass">, "error out"=w297:errorcluster)  [unwired: 15 in]
          n119 = call-dynamic "ManageInterfaces.vi"("ClassWriter.lvclass"=w298, "ClassRef"=w294, "HandleInterfacesData"=w293, "error in (no error)"=w297) -> ("ClassWriter.lvclass"=w295:refnum<class "ClassWriter.lvclass">, "error out"=w296:errorcluster)  [unwired: 14 in]
        }
        frame True {
        }
      }
      n120 = call-dynamic "Destroy.vi"("ClassWriter.lvclass"=w286, "error in (no error)"=w287) -> ("error out"=w288:errorcluster)  [unwired: 17 in]
      n121 = Close Reference(reference=w279, error in (no error)=w288) -> (error out=w292:errorcluster)
      n122 = Close Reference(reference=w271, error in (no error)=w292) -> (error out=w284:errorcluster)
      n123 = call <resource>:"GDSError_ReportError.vi"("error in (no error)"=w284) -> ()  [unwired: 18 in, 1 out]
    }
    frame "ModifyInheritance" {
      w318 = refnum<vi> refnum  # LVClassLibrary
      # "Not allowed"
      n124 = call <resource>:"GOOP_GetClassProvider.vi"("New Item Parent/Object"=w323, "ProviderClassType"=GOOP_ClassProviderClassType."ClassWriter") -> ("ProjectItem"=w319:refnum<vi>, "LVClass.Open"=w310:refnum<vi>, "error out"=w309:errorcluster)  [unwired: 15 in]
      n125 = To More Specific Class(target class=w318, reference=w319) -> (specific class reference=w304:refnum<vi>)  [unwired: 1 in, 1 out]
      n126 = call <resource>:"GOOP_GetDefaultInstance.vi"("error in"=w309, "LVClassIn"=w310) -> ("error out"=w305:errorcluster, "ClassWriter.lvclass"=w308:refnum<class "ClassWriter.lvclass">, "LVClassOut"=w311:refnum<vi>)  [unwired: 7 in]
      n127 = call-dynamic "Init.vi"("ClassWriter in"=w308, "error in (no error)"=w305, "LVClassLibrary Refnum"=w304) -> ("ClassWriter out"=w307:refnum<class "ClassWriter.lvclass">, "error out"=w306:errorcluster)  [unwired: 15 in]
      n128 = call-dynamic "ChangeInheritanceDialog.vi"("ClassWriter in"=w307, "LvClass"=w304, "error in (no error)"=w306) -> ("ClassWriter out"=w316:refnum<class "ClassWriter.lvclass">, "BaseClassPath"=w312:path, "Cancelled"=w313:bool, "error out"=w315:errorcluster)  [unwired: 13 in]
      n129 = case shown="False" w313 {
        tunnel: w316 -> [w325 _]
        tunnel: w315 -> [w327 w334]
        tunnel: [w333 w334] -> w314
        tunnel: w304 -> [w332 _]
        tunnel: w312 -> [w331 _]
        frame False {
          n130 = call <resource>:"GdsLanguage_GetTranslatedString.vi"("StringID(s)"="ChangeingInheritanceStatusMessage" ("Message(Exit)"), "error in (no error)"=w327) -> ("FirstStringOut"=w328:string, "error out"=w329:errorcluster)  [unwired: 14 in, 2 out]
          n131 = call-dynamic "ProgressWindow.vi"("ClassWriter in"=w325, "Message(Exit)"=w328, "error in (no error)"=w329) -> ("ClassWriter out"=w324:refnum<class "ClassWriter.lvclass">, "error out"=w326:errorcluster)  [unwired: 15 in]
          n132 = call-dynamic "ChangeInheritance.vi"("ClassWriter in"=w324, "LvClass"=w332, "NewBaseClass(Empty=ConvertClassToBaseClass)"=w331, "error in (no error)"=w326) -> ("error out"=w333:errorcluster)  [unwired: 14 in, 1 out]
        }
        frame True {
        }
      }
      n133 = call-dynamic "Destroy.vi"("ClassWriter.lvclass"=w307, "error in (no error)"=w314) -> ("error out"=w317:errorcluster)  [unwired: 17 in]
      n134 = Close Reference(reference=w311, error in (no error)=w317) -> (error out=w322:errorcluster)
      n135 = Close Reference(reference=w304, error in (no error)=w322) -> (error out=w321:errorcluster)
      n136 = call <resource>:"GDSError_ReportError.vi"("error in (no error)"=w321) -> ()  [unwired: 18 in, 1 out]
    }
    frame "RenameClass" {
      w355 = refnum<vi> refnum  # LVClassLibrary
      # "Not allowed"
      n137 = call <resource>:"GOOP_GetClassProvider.vi"("New Item Parent/Object"=w347, "ProviderClassType"=GOOP_ClassProviderClassType."ClassWriter") -> ("ProjectItem"=w356:refnum<vi>, "LVClass.Open"=w338:refnum<vi>, "error out"=w339:errorcluster)  [unwired: 15 in]
      n138 = To More Specific Class(target class=w355, reference=w356) -> (specific class reference=w341:refnum<vi>)  [unwired: 1 in, 1 out]
      n139 = call <resource>:"GOOP_GetDefaultInstance.vi"("error in"=w339, "LVClassIn"=w338) -> ("error out"=w336:errorcluster, "ClassWriter.lvclass"=w337:refnum<class "ClassWriter.lvclass">, "LVClassOut"=w335:refnum<vi>)  [unwired: 7 in]
      n140 = call-dynamic "Init.vi"("ClassWriter in"=w337, "error in (no error)"=w336, "LVClassLibrary Refnum"=w341) -> ("ClassWriter out"=w345:refnum<class "ClassWriter.lvclass">, "error out"=w344:errorcluster)  [unwired: 15 in]
      n141 = call <resource>:"CheckThatClassIsWritable.vi"("ClassWriter in"=w345, "Library Refnum"=w341, "error in (no error)"=w344) -> ("ClassWriter out"=w343:refnum<class "ClassWriter.lvclass">, "error out"=w342:errorcluster)  [unwired: 15 in]
      n142 = call-dynamic "DialogRenameClass.vi"("ClassWriter.lvclass"=w343, "ClassItemRefIn"=w341, "error in (no error)"=w342) -> ("ClassWriter.lvclassOut"=w353:refnum<class "ClassWriter.lvclass">, "NewClassPath"=w349:path, "Cancelled"=w350:bool, "RelinkWholeProject"=w340:bool, "error out"=w352:errorcluster)  [unwired: 11 in, 1 out]
      n143 = case shown="False" w350 {
        tunnel: w353 -> [w366 w371]
        tunnel: w352 -> [w363 w372]
        tunnel: [w367 w372] -> w351
        tunnel: w341 -> [w370 _]
        tunnel: w349 -> [w369 _]
        tunnel: [w368 w371] -> w348
        tunnel: w340 -> [w359 _]
        frame False {
          n144 = call <resource>:"GdsLanguage_GetTranslatedString.vi"("StringID(s)"="RenamingClassStatusMessage" ("Message(Exit)"), "error in (no error)"=w363) -> ("FirstStringOut"=w360:string, "error out"=w362:errorcluster)  [unwired: 14 in, 2 out]
          n145 = call-dynamic "ProgressWindow.vi"("ClassWriter in"=w366, "Message(Exit)"=w360, "error in (no error)"=w362) -> ("ClassWriter out"=w365:refnum<class "ClassWriter.lvclass">, "error out"=w364:errorcluster)  [unwired: 15 in]
          n146 = call-dynamic "RenameClass.vi"("ClassWriter.lvclass"=w365, "ClassRef"=w370, "NewClassPath"=w369, "RelinkWholeProject"=w359, "error in (no error)"=w364) -> ("ClassWriter.lvclass"=w368:refnum<class "ClassWriter.lvclass">, "error out"=w367:errorcluster)  [unwired: 13 in]
        }
        frame True {
        }
      }
      n147 = call-dynamic "Destroy.vi"("ClassWriter.lvclass"=w348, "error in (no error)"=w351) -> ("error out"=w354:errorcluster)  [unwired: 17 in]
      n148 = Close Reference(reference=w335, error in (no error)=w354) -> (error out=w358:errorcluster)
      n149 = Close Reference(reference=w341, error in (no error)=w358) -> (error out=w346:errorcluster)
      n150 = call <resource>:"GDSError_ReportError.vi"("error in (no error)"=w346) -> ()  [unwired: 18 in, 1 out]
    }
    frame "UmlViewClass" {
      # "OK to do"
      n151 = call <resource>:"mxLvGetItemRef.vi"("Item"=w373) -> ("Item Refnum"=w375:refnum<vi>, "error out"=w385:errorcluster)  [unwired: 1 in, 1 out]
      n152 = property class="ProjectItem"(reference=w375, error in=w385) -> (reference out=w381:refnum<vi>, error out=w401:errorcluster, "Project"=w376:refnum<vi>, "Type String"=w383:string, "Target"=w397:refnum<vi>)
      n153 = property class="TargetItem"(reference=w397, error in=w401) -> (reference out=w399:refnum<vi>, error out=w400:errorcluster, "Name"=w398:string)
      n154 = case shown="Default" w383 {
        tunnel: w381 -> [w402 w408 w414]
        tunnel: [w402 w404 w410] -> w382
        tunnel: [_ w403 w409] -> w384
        frame Default {
        }
        frame "LvClass" {
          w407 = refnum<vi> refnum  # LVClassLibrary
          n155 = To More Specific Class(target class=w407, reference=w408) -> (specific class reference=w406:refnum<vi>, error out=w405:errorcluster)  [unwired: 1 in]
          n156 = property class="LVClassLibrary"(reference=w406, error in=w405) -> (reference out=w404:refnum<vi>, "Path"=w403:path)  [unwired: 1 out]
        }
        frame "VI" {
          w413 = refnum<vi> refnum  # ProjectItem
          n157 = To More Specific Class(target class=w413, reference=w414) -> (specific class reference=w412:refnum<vi>, error out=w411:errorcluster)  [unwired: 1 in]
          n158 = property class="ProjectItem"(reference=w412, error in=w411) -> (reference out=w410:refnum<vi>, "Path"=w409:path)  [unwired: 1 out]
        }
      }
      n159 = property class="Project"(reference=w376, error in=w401) -> (reference out=w379:refnum<vi>, error out=w378:errorcluster, "Name"=w377:string)
      n160 = Close Reference(reference=w399, error in (no error)=w400) -> ()  [unwired: 1 out]
      n161 = Close Reference(reference=w379, error in (no error)=w378) -> (error out=w380:errorcluster)
      n162 = Close Reference(reference=w382, error in (no error)=w380) -> (error out=w389:errorcluster)
      n163 = call-dynamic "Init.vi"("ClassWriter in"=refnum<class "ClassWriter.lvclass"> refnum, "error in (no error)"=w389) -> ("ClassWriter out"=w394:refnum<class "ClassWriter.lvclass">, "error out"=w390:errorcluster)  [unwired: 16 in]
      n164 = call <resource>:"GdsLanguage_GetTranslatedString.vi"("StringID(s)"="UmlViewClasses" ("Message(Exit)"), "error in (no error)"=w390) -> ("FirstStringOut"=w386:string, "error out"=w387:errorcluster)  [unwired: 14 in, 2 out]
      n165 = call-dynamic "ProgressWindow.vi"("ClassWriter in"=w394, "Message(Exit)"=w386, "error in (no error)"=w387) -> ("ClassWriter out"=w393:refnum<class "ClassWriter.lvclass">, "error out"=w391:errorcluster)  [unwired: 15 in]
      n166 = call <resource>:"GOOP_UMLEditor_CallMain.vi"("Enum"=GOOP_UMLEditor_CallMainAction."ReverseEngineering:OneClass", "Project"=w377, "Class/VI-Path"=w384, "Target"=w398, "error in (no error)"=w391) -> ("error out"=w392:errorcluster)  [unwired: 14 in]
      n167 = call-dynamic "Destroy.vi"("ClassWriter.lvclass"=w393, "error in (no error)"=w392) -> ("error out"=w395:errorcluster)  [unwired: 17 in]
      n168 = call <resource>:"GDSError_ReportError.vi"("error in (no error)"=w395) -> ()  [unwired: 18 in, 1 out]
    }
    frame "UpdateMessageClass" {
      w452 = refnum<vi> refnum  # LVClassLibrary
      # "From Message Class Ref\nGet Actor method"
      # "Not allowed"
      n169 = call <resource>:"mxLvGetItemRef.vi"("Item"=w451) -> ("Item Refnum"=w450:refnum<vi>, "error out"=w426:errorcluster)  [unwired: 1 in, 1 out]
      n170 = call-dynamic "Init.vi"("ClassWriter in"=refnum<class "ClassWriter.lvclass"> refnum, "error in (no error)"=w426) -> ("ClassWriter out"=w420:refnum<class "ClassWriter.lvclass">, "error out"=w423:errorcluster)  [unwired: 16 in]
      n171 = call <resource>:"GdsLanguage_GetTranslatedString.vi"("StringID(s)"="UpdateMessageClass" ("Message(Exit)"), "error in (no error)"=w423) -> ("FirstStringOut"=w424:string, "error out"=w422:errorcluster)  [unwired: 14 in, 2 out]
      n172 = disable-structure shown="Enabled" {
        disable-tunnel: w424 -> [w457 _]
        disable-tunnel: [w456 w459] -> w417
        disable-tunnel: w422 -> [w455 w459]
        disable-tunnel: w420 -> [w454 w458]
        disable-tunnel: [w453 w458] -> w419
        frame Enabled {
          n173 = call-dynamic "ProgressWindow.vi"("ClassWriter in"=w454, "Message(Exit)"=w457, "error in (no error)"=w455) -> ("ClassWriter out"=w453:refnum<class "ClassWriter.lvclass">, "error out"=w456:errorcluster)  [unwired: 15 in]
        }
        frame Disabled {
        }
      }
      n174 = To More Specific Class(target class=w452, reference=w450) -> (specific class reference=w416:refnum<vi>)  [unwired: 1 in, 1 out]
      n175 = property class="LVClassLibrary"(reference=w416, error in=w417) -> (error out=w448:errorcluster, "Project"=w447:refnum<vi>, "Path"=w444:path)  [unwired: 1 out]
      n176 = property class="Project"(reference=w447, error in=w448) -> (error out=w437:errorcluster, "App Ref"=w446:refnum<vi>)  [unwired: 1 out]
      n177 = invoke class="LVClassLibrary" method="Get All Descendents"(reference=w416, error in=w437, "Type"="VI") -> (error out=w439:errorcluster, "All Descendents"=w431:refnum<vi>[])  [unwired: 4 in, 5 out]
      n178 = for {
        tunnel: w431 -> [w467] mode=indexing
        tunnel: [w463] -> w441
        shift-right: [w462] -> w440
        shift-left: w439 -> [w461]
        stop <- w460 stop-if-true
        n179 = property class="ProjectItem"(reference=w467, error in=w461) -> (reference out=w463:refnum<vi>, error out=w462:errorcluster, "Name"=w466:string)
        n180 = To Lower Case(string=w466) -> (all lower case string=w465:string)
        n181 = Equal?(x=w465, y="do.vi") -> (x = y?=w460:bool)
      }
      n182 = Strip Path(path=w444) -> (stripped path=w443:path)  [unwired: 1 out]
      n183 = property class="ProjectItem"(reference=w441, error in=w440) -> (error out=w435:errorcluster, "Reference"=w438:refnum<vi>)  [unwired: 1 out]
      n184 = invoke class="VI" method="Get VI Dependencies"(reference=w438, error in=w435, "Dynamic Dispatching?"=T3."Include nearest implementation") -> (reference out=w433:refnum<vi>, error out=w434:errorcluster, "Dependency Paths"=w430:path[])  [unwired: 16 in, 16 out]
      n185 = Close Reference(reference=w433, error in (no error)=w434) -> (error out=w432:errorcluster)
      n186 = Index Array(array=w430) -> (element=w429:path)  [unwired: 1 in]
      n187 = Close Reference(reference=w431, error in (no error)=w432) -> (error out=w428:errorcluster)
      n188 = call <resource>:"MM.vi"("AppInst"=w446, "ActorMethod"=w429, "ActorClassItemRef(Don't Delete)"=refnum<vi> refnum, "OnlyUpdate(if needed,False)"=TRUE ("OnlyUpdate(if needed)"), "Destination Path"=w443, "error in"=w428) -> ("error out"=w427:errorcluster)  [unwired: 13 in]
      n189 = Close Reference(reference=w416, error in (no error)=w427) -> (error out=w449:errorcluster)
      n190 = call <resource>:"GDSError_ReportError.vi"("error in (no error)"=w449) -> ("error out"=w421:errorcluster)  [unwired: 18 in]
      n191 = call-dynamic "Destroy.vi"("ClassWriter.lvclass"=w419, "error in (no error)"=w421) -> ()  [unwired: 17 in, 1 out]
    }
    frame "UpdateMessageClasses" {
      w495 = refnum<vi> refnum  # LVClassLibrary
      # "From Message Class Ref\nGet Actor method"
      n192 = call <resource>:"mxLvGetItemRef.vi"("Item"=w470) -> ("Item Refnum"=w494:refnum<vi>, "error out"=w475:errorcluster)  [unwired: 1 in, 1 out]
      n193 = To More Specific Class(target class=w495, reference=w494, error in=w475) -> (specific class reference=w469:refnum<vi>, error out=w474:errorcluster)
      n194 = call-dynamic "Init.vi"("ClassWriter in"=refnum<class "ClassWriter.lvclass"> refnum, "error in (no error)"=w474) -> ("ClassWriter out"=w477:refnum<class "ClassWriter.lvclass">, "error out"=w479:errorcluster)  [unwired: 16 in]
      n195 = call <resource>:"GdsLanguage_GetTranslatedString.vi"("StringID(s)"="UpdateMessageClass" ("Message(Exit)"), "error in (no error)"=w479) -> ("FirstStringOut"=w480:string, "error out"=w478:errorcluster)  [unwired: 14 in, 2 out]
      n196 = disable-structure shown="Enabled" {
        disable-tunnel: w480 -> [w500 _]
        disable-tunnel: [w499 w502] -> w468
        disable-tunnel: w478 -> [w498 w502]
        disable-tunnel: w477 -> [w497 w501]
        disable-tunnel: [w496 w501] -> w471
        frame Enabled {
          n197 = call-dynamic "ProgressWindow.vi"("ClassWriter in"=w497, "Message(Exit)"=w500, "error in (no error)"=w498) -> ("ClassWriter out"=w496:refnum<class "ClassWriter.lvclass">, "error out"=w499:errorcluster)  [unwired: 15 in]
        }
        frame Disabled {
        }
      }
      n198 = property class="LVClassLibrary"(reference=w469, error in=w468) -> (reference out=w487:refnum<vi>, error out=w492:errorcluster, "Project"=w493:refnum<vi>)
      n199 = property class="Project"(reference=w493, error in=w492) -> (reference out=w488:refnum<vi>, error out=w489:errorcluster, "App Ref"=w491:refnum<vi>)
      n200 = invoke class="LVClassLibrary" method="Get All Descendents"(reference=w487, error in=w489, "Type"="VI") -> (reference out=w484:refnum<vi>, error out=w485:errorcluster, "All Descendents"=w482:refnum<vi>[])  [unwired: 4 in, 4 out]
      n201 = for {
        tunnel: w491 -> [w510]
        shift-right: [w504] -> w483
        shift-left: w485 -> [w507]
        tunnel: w482 -> [w508] mode=indexing
        tunnel: w484 -> [w509]
        tunnel: w469 -> [w503]
        stop <- w504 stop-if-true
        n202 = invoke class="LVClassLibrary" method="Get Source Scope"(reference=w509, error in=w507, "SourceRef"=w508) -> (error out=w506:errorcluster, "GetSourceScope"=w505:T16)  [unwired: 2 in, 3 out]
        n203 = case shown="\"public\", Default" w505 {
          tunnel: [w511 w519] -> w504
          tunnel: w510 -> [_ w518]
          tunnel: w508 -> [_ w515]
          tunnel: w506 -> [w511 w514]
          tunnel: w503 -> [_ w512]
          frame "private", "protected" {
          }
          frame "public", Default {
            n204 = property class="ProjectItem"(reference=w515, error in=w514) -> (error out=w516:errorcluster, "Path"=w517:path)  [unwired: 1 out]
            n205 = call <resource>:"MM.vi"("AppInst"=w518, "ActorMethod"=w517, "ActorClassItemRef(Don't Delete)"=w512, "OnlyUpdate(if needed,False)"=FALSE, "error in"=w516) -> ("error out"=w519:errorcluster)  [unwired: 14 in]
          }
        }
      }
      n206 = Close Reference(reference=w482, error in (no error)=w483) -> ()  [unwired: 1 out]
      n207 = Close Reference(reference=w491, error in (no error)=w483) -> (error out=w490:errorcluster)
      n208 = Close Reference(reference=w488, error in (no error)=w490) -> (error out=w473:errorcluster)
      n209 = call-dynamic "Destroy.vi"("ClassWriter.lvclass"=w471, "error in (no error)"=w473) -> ("error out"=w472:errorcluster)  [unwired: 17 in]
      n210 = call <resource>:"GDSError_ReportError.vi"("error in (no error)"=w472) -> ()  [unwired: 18 in, 1 out]
    }
    frame Default {
      n211 = Match Pattern(string=w522, regular expression="\\2E[Pp][Nn][Gg]") -> (before substring=w520:string, offset past match=w521:i32)  [unwired: 1 in, 2 out]
      n212 = case shown="Default" w521 {
        tunnel: w523 -> [w525 _]
        tunnel: w522 -> [_ _]
        tunnel: w520 -> [w526 _]
        frame Default {
          w532 = refnum<vi> refnum  # LVClassLibrary
          n213 = call <resource>:"mxLvGetItemRef.vi"("Item"=w525) -> ("Item Refnum"=w531:refnum<vi>, "error out"=w530:errorcluster)  [unwired: 1 in, 1 out]
          n214 = call <resource>:"GOOP_ApplyOverlayIcon.vi"("error in (no error)"=w530, "IconName(NoPngExtension)"=w526, "Object"=w525) -> ("error out"=w529:errorcluster)  [unwired: 8 in]
          n215 = To More Specific Class(target class=w532, reference=w531) -> (specific class reference=w528:refnum<vi>)  [unwired: 1 in, 1 out]
          n216 = call <resource>:"GDSLvClass_StoreClassItemIcon.vi"("Library Refnum"=w528, "ClassItemIconName"=w526, "error in (no error)"=w529) -> ("error out"=w527:errorcluster)  [unwired: 15 in, 1 out]
          n217 = Close Reference(reference=w528, error in (no error)=w527) -> ()  [unwired: 1 out]
        }
        frame -1 {
        }
      }
    }
  }
